vi "FuncVI_Sub - Probe - Launcher.vi"(8 "error in":errorcluster, 9 "left-top corner":cluster{"x":i16, "y":i16}={"x"=-1, "y"=-1}, 10 "win name":string, 11 "arg":T1) -> (0 "error out":errorcluster)   [LabVIEW 2021]
doc: "::: CalcExpress Toolkit :::\nCopyright (c) 2000-2026 Konstantin Shifershteyn. All rights reserved."
uses:
  cetypes.llb/CalcExpress Function Argument Info.ctl
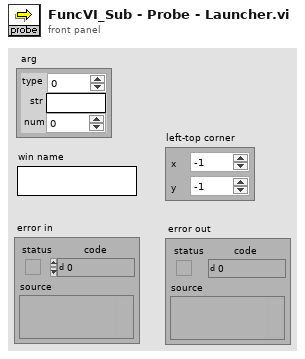
[diagram p1: front panel]
types:
  T1 = typedef "CalcExpress Function Argument Info.ctl" = cluster{"type":u32, "str":string, "num":dbl}
  T2 = enum32{"Invalid", "Standard", "Closed", "Hidden", "Minimized", "Maximized"}
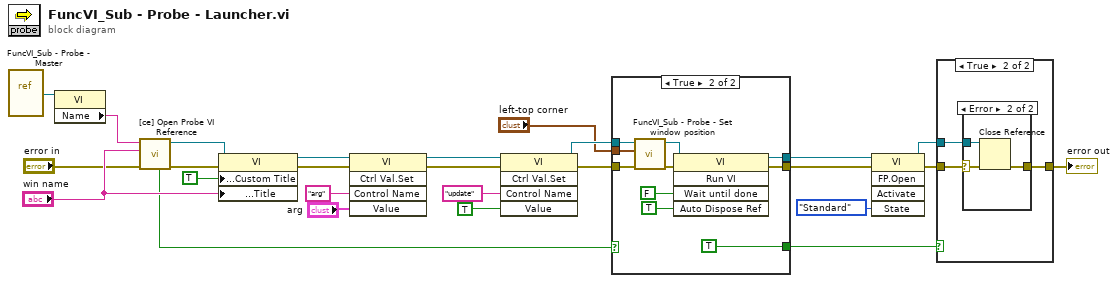
[diagram p0: block diagram]
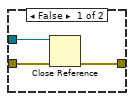
[diagram p2: hidden frame]
diagram:
  n1 = vi-ref "FuncVI_Sub - Probe - Master.vi"() -> (w6:refnum<vi>)
  n2 = property class="VI"(reference=w6) -> ("Name"=w5:string)  [unwired: 1 in, 2 out]
  n3 = call "[ce] Open Probe VI Reference.vi"("error in"="error in", "VI instance name"="win name", "master VI name"=w5) -> ("error out"=w14:errorcluster, "vi refnum"=w13:refnum<vi>, "new window?"=w11:bool)  [unwired: 6 in]
  n4 = property class="VI"(reference=w13, error in=w14, "Front Panel Window:Custom Title"=TRUE ("Front Panel.CustomTitle"), "Front Panel Window:Title"="win name") -> (reference out=w16:refnum<vi>, error out=w15:errorcluster)
  n5 = invoke class="VI" method="Ctrl Val.Set"(reference=w16, error in=w15, "Control Name"="arg", "Value"="arg") -> (reference out=w21:refnum<vi>, error out=w20:errorcluster)  [unwired: 1 in, 3 out]
  n6 = invoke class="VI" method="Ctrl Val.Set"(reference=w21, error in=w20, "Control Name"="update", "Value"=TRUE) -> (reference out=w19:refnum<vi>, error out=w18:errorcluster)  [unwired: 1 in, 3 out]
  n7 = case shown="True" w11 {
    tunnel: [w28 w36] -> w25
    tunnel: [w27 w37] -> w24
    tunnel: w19 -> [w28 w32]
    tunnel: w18 -> [w27 w35]
    tunnel: [_ TRUE] -> w2
    tunnel: "left-top corner" -> [_ w29]
    frame False {
    }
    frame True {
      n8 = call "FuncVI_Sub - Probe - Set window position.vi"("error in"=w35, "left-top corner"=w29, "VI RefNum"=w32) -> ("error out"=w34:errorcluster, "dup VI Refnum"=w33:refnum<vi>)  [unwired: 7 in]
      n9 = invoke class="VI" method="Run VI"(reference=w33, error in=w34, "Wait until done"=FALSE, "Auto Dispose Ref"=TRUE ("Auto Dispose Reference")) -> (reference out=w36:refnum<vi>, error out=w37:errorcluster)  [unwired: 1 in, 3 out]
    }
  }
  n10 = invoke class="VI" method="FP.Open"(reference=w25, error in=w24, "State"=T2."Standard") -> (reference out=w26:refnum<vi>, error out=w4:errorcluster)  [unwired: 2 in, 3 out]
  n11 = case shown="True" w2 {
    tunnel: w26 -> [w41 w44]
    tunnel: w4 -> [w40 w43]
    tunnel: [w39 w42] -> w3
    frame False {
      n12 = Close Reference(reference=w41, error in (no error)=w40) -> (error out=w39:errorcluster)
    }
    frame True {
      n13 = case shown="Error" w43 {
        selector: w43 -> [w45 w47]
        tunnel: w44 -> [_ w48]
        tunnel: [w45 w46] -> w42
        frame No Error {
        }
        frame Error {
          n14 = Close Reference(reference=w48, error in (no error)=w47) -> (error out=w46:errorcluster)
        }
      }
    }
  }
  "error out" <- w3
